vi "Exo_interfaces.vi"() -> ()   [LabVIEW 2012]
uses:
  Control 1.ctl
panel:
  in  "stop":bool
  out "message":string
  out "y":dbl
  in  "b 2":i32
  in  "A":i32
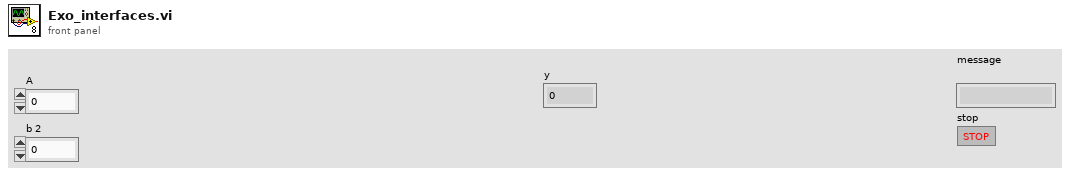
[diagram p1: front panel]
types:
  T1 = typedef "Control 1.ctl" = string
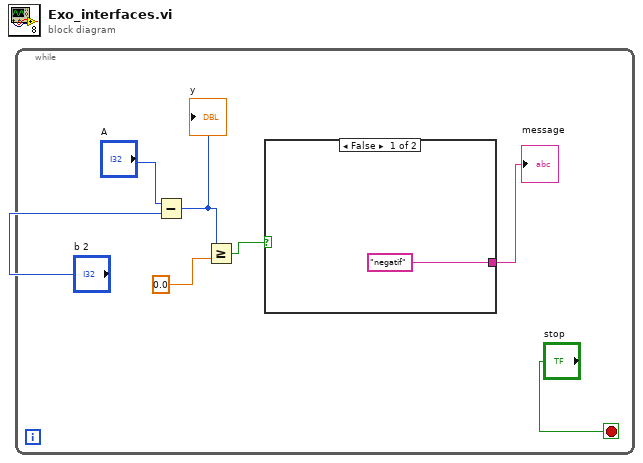
[diagram p0: block diagram]
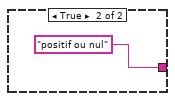
[diagram p2: hidden frame]
diagram:
  n1 = while {
    stop <- "stop" stop-if-true
    n2 = Subtract(x="A", y="b 2") -> (x-y=w3:i32)
    "y" <- w3
    n3 = Greater Or Equal?(x=w3, y=0.0) -> (x >= y?=w4:bool)
    n4 = case shown="False" w4 {
      tunnel: ["negatif" T1 "positif ou nul"] -> w2
      frame False {
      }
      frame True {
      }
    }
    "message" <- w2
  }
